vi "Sample.vi"(8 "错误输入（无错误）":errorcluster, 9 "Calib(+)":dbl[](array[numeric]), 10 "VISA资源名称":refnum<visa-resource-name>) -> (0 "error out":errorcluster, 2 "Data Out":dbl[](array[numeric]) format="%.2f")   [LabVIEW 2026, in "UI-温度采集.lvlib" / "Acquisition.lvlib"]
uses:
  Acquisition.lvlib
  a24846f6-4cfe-4367-9c5b-2cc2081cb94c.vi
  <vilib>/ptbypt/NI_PtbyPt.lvlib
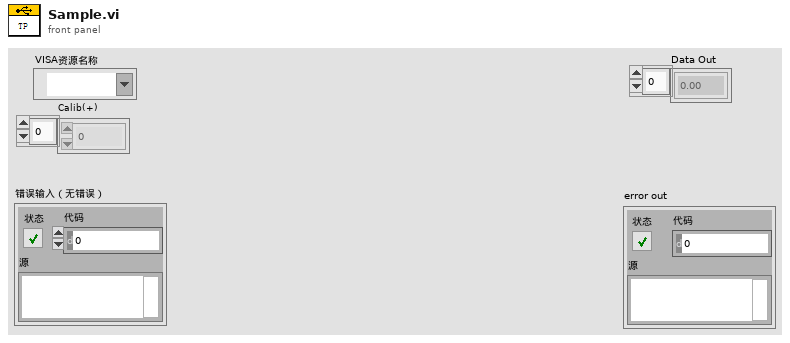
[diagram p1: front panel]
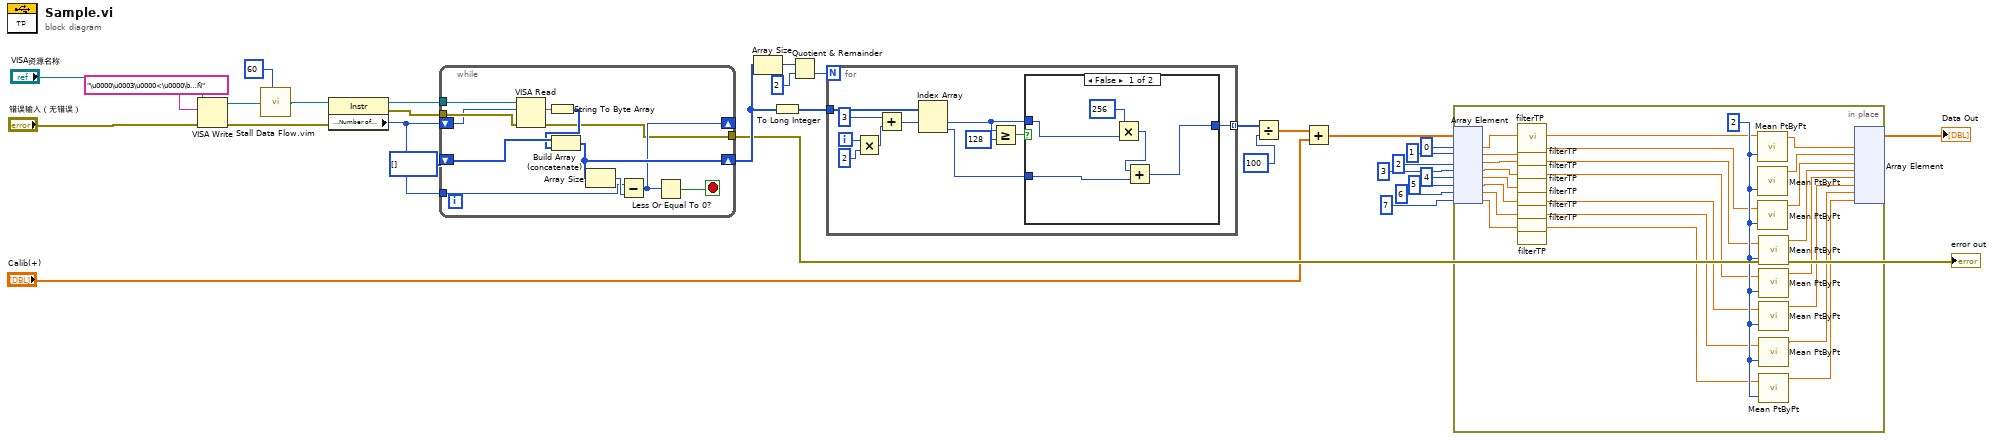
[diagram p0: block diagram]
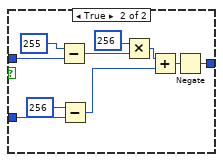
[diagram p2: hidden frame]
diagram:
  n1 = VISA Write(VISA resource name="VISA资源名称", write buffer="\u0000\u0003\u0000<\u0000\b…Ñ" ("Command"), error in (no error)="错误输入（无错误）") -> (VISA resource name out=w2:refnum<visa-resource-name>, error out=w4:errorcluster)  [unwired: 1 out]
  n2 = call "Stall Data Flow.vim"("value in"=w2, "milliseconds to wait"=u32 60 ("读取前延时(ms)")) -> ("value out"=w3:refnum<visa-resource-name>)  [unwired: 1 out]
  n3 = property class="Instr"(reference=w3, error in=w4) -> (reference out=w24:refnum<visa-resource-name>, error out=w23:errorcluster, "Serial Settings:Number of Bytes at Serial Port"=w22:u32)
  n4 = while {
    tunnel: w24 -> [w41]
    tunnel: w23 -> [w40]
    shift-right: [w43] -> w29
    shift-left: u8[] [] ("unsigned byte array") -> [w42]
    tunnel: w22 -> [w35]
    shift-right: [w33] -> _
    shift-left: w22 -> [w39]
    tunnel: [w32] -> w17
    stop <- w34 stop-if-true
    n5 = VISA Read(VISA resource name=w41, byte count=w39, error in (no error)=w40) -> (read buffer=w38:string, error out=w32:errorcluster)  [unwired: 2 out]
    n6 = String To Byte Array(string=w38) -> (unsigned byte array=w37:u8[])
    n7 = Build Array (concatenate)(w42, w37) -> (w43:u8[])
    n8 = Array Size(array=w43) -> (size(s)=w36:i32)
    n9 = Subtract(x=w35, y=w36) -> (x-y=w33:u32)
    n10 = Less Or Equal To 0?(x=w33) -> (x <= 0?=w34:bool)
  }
  "error out" <- w17
  n11 = Array Size(array=w29) -> (size(s)=w27:i32)
  n12 = To Long Integer(number=w29) -> (32bit integer=w30:i32[])
  n13 = Quotient & Remainder(x=w27, y=2) -> (floor(x/y)=w26:i32)  [unwired: 1 out]
  n14 = for {
    N: w26 -> [_]
    tunnel: w30 -> [w54]
    tunnel: [w44] -> w18 mode=indexing
    i -> [w51]
    n15 = Multiply(x=w51, y=2) -> (x*y=w49:i32)
    n16 = Add(x=3 ("索引"), y=w49) -> (x+y=w52:i32)
    n17 = Index Array(array=w54, index #1=w52) -> (element #1=w46:i32, element #2=w45:i32)  [unwired: 1 in]
    n18 = Greater Or Equal?(x=w46, y=128) -> (x >= y?=w48:bool)
    n19 = case shown="False" w48 {
      tunnel: w46 -> [w58 w67]
      tunnel: w45 -> [w56 w65]
      tunnel: [w55 w60] -> w44
      frame False {
        n20 = Multiply(x=256, y=w58) -> (x*y=w59:i32)
        n21 = Add(x=w59, y=w56) -> (x+y=w55:i32)
      }
      frame True {
        n22 = Subtract(x=255, y=w67) -> (x-y=w64:i32)
        n23 = Subtract(x=256, y=w65) -> (x-y=w62:i32)
        n24 = Multiply(x=256, y=w64) -> (x*y=w63:i32)
        n25 = Add(x=w63, y=w62) -> (x+y=w61:i32)
        n26 = Negate(x=w61) -> (-x=w60:i32)
      }
    }
  }
  n27 = Divide(x=w18, y=100) -> (x/y=w16:dbl[])
  n28 = Add(x=w16, y="Calib(+)") -> (x+y=w14:dbl[])
  n29 = in-place {
    w93 = 2 ("sample length")
    n30 = in-place-array #1(w14, 0, 1, 2, 3, 4, 5, 6, 7) -> (w84:dbl, w82:dbl, w80:dbl, w78:dbl, w76:dbl, w75:dbl, w73:dbl, w71:dbl)
    n31 = call "filterTP.vi"("输入"=w84) -> ("输出"=w83:dbl)  [unwired: 10 in]
    n32 = call "filterTP.vi"("输入"=w82) -> ("输出"=w81:dbl)  [unwired: 10 in]
    n33 = call "filterTP.vi"("输入"=w80) -> ("输出"=w79:dbl)  [unwired: 10 in]
    n34 = call "filterTP.vi"("输入"=w78) -> ("输出"=w77:dbl)  [unwired: 10 in]
    n35 = call "filterTP.vi"("输入"=w76) -> ()  [unwired: 10 in, 1 out]
    n36 = call "filterTP.vi"("输入"=w75) -> ("输出"=w74:dbl)  [unwired: 10 in]
    n37 = call "filterTP.vi"("输入"=w73) -> ("输出"=w72:dbl)  [unwired: 10 in]
    n38 = call "filterTP.vi"("输入"=w71) -> ("输出"=w70:dbl)  [unwired: 10 in]
    n39 = call <vilib>:"Mean PtByPt.vi"("x"=w83, "sample length"=w93) -> ("mean"=w92:dbl)  [unwired: 2 in, 1 out]
    n40 = call <vilib>:"Mean PtByPt.vi"("sample length"=w93) -> ("mean"=w91:dbl)  [unwired: 3 in, 1 out]
    n41 = call <vilib>:"Mean PtByPt.vi"("x"=w81, "sample length"=w93) -> ("mean"=w90:dbl)  [unwired: 2 in, 1 out]
    n42 = call <vilib>:"Mean PtByPt.vi"("x"=w79, "sample length"=w93) -> ("mean"=w89:dbl)  [unwired: 2 in, 1 out]
    n43 = call <vilib>:"Mean PtByPt.vi"("x"=w77, "sample length"=w93) -> ("mean"=w88:dbl)  [unwired: 2 in, 1 out]
    n44 = call <vilib>:"Mean PtByPt.vi"("x"=w74, "sample length"=w93) -> ("mean"=w87:dbl)  [unwired: 2 in, 1 out]
    n45 = call <vilib>:"Mean PtByPt.vi"("x"=w72, "sample length"=w93) -> ("mean"=w86:dbl)  [unwired: 2 in, 1 out]
    n46 = call <vilib>:"Mean PtByPt.vi"("x"=w70, "sample length"=w93) -> ("mean"=w85:dbl)  [unwired: 2 in, 1 out]
    n47 = in-place-array #1(w92, w91, w90, w89, w88, w87, w86, w85) -> (→"Data Out":dbl[])  [unwired: 8 out]
  }
